vi "monitor registers.vi"(7 "register monitor queue":refnum<queue>, 8 "error in":errorcluster, 9 "Registers":T1[](array[typedef]), 10 "bus instance name":string, 11 "fpga interface in":refnum<k20>) -> (0 "error out":errorcluster, 2 "registers out":string[][](array[string]), 3 "fpga interface out":refnum<k20>, 5 "register monitor queue out":refnum<queue>)   [LabVIEW 2025, in "Automotive Vision.lvclass"]
uses:
  Automotive Vision.lvclass
  Automotive Vision.lvclass/Automotive Vision.ctl
  <instrlib>/FlexRIO/API/Host/v1/NI FlexRIO API v1.lvlib
  regitster_value.ctl
  register.ctl
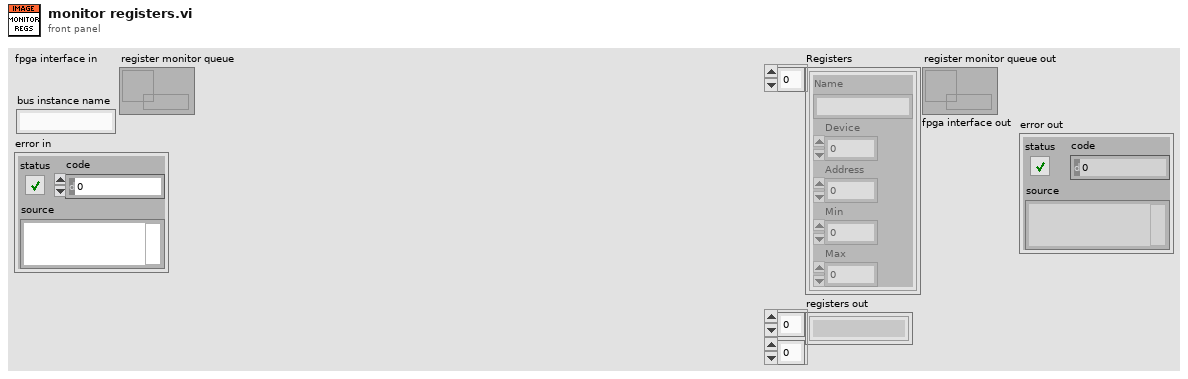
[diagram p1: front panel]
types:
  T1 = typedef "Automotive Vision.lvclass/register.ctl" = cluster{"Name":string, "Device":u8, "Address":u16, "Min":u16, "Max":u16}
  T2 = typedef "Automotive Vision.lvclass/regitster_value.ctl" = cluster{"Source":u8, "Address":u16, "Value":u16}
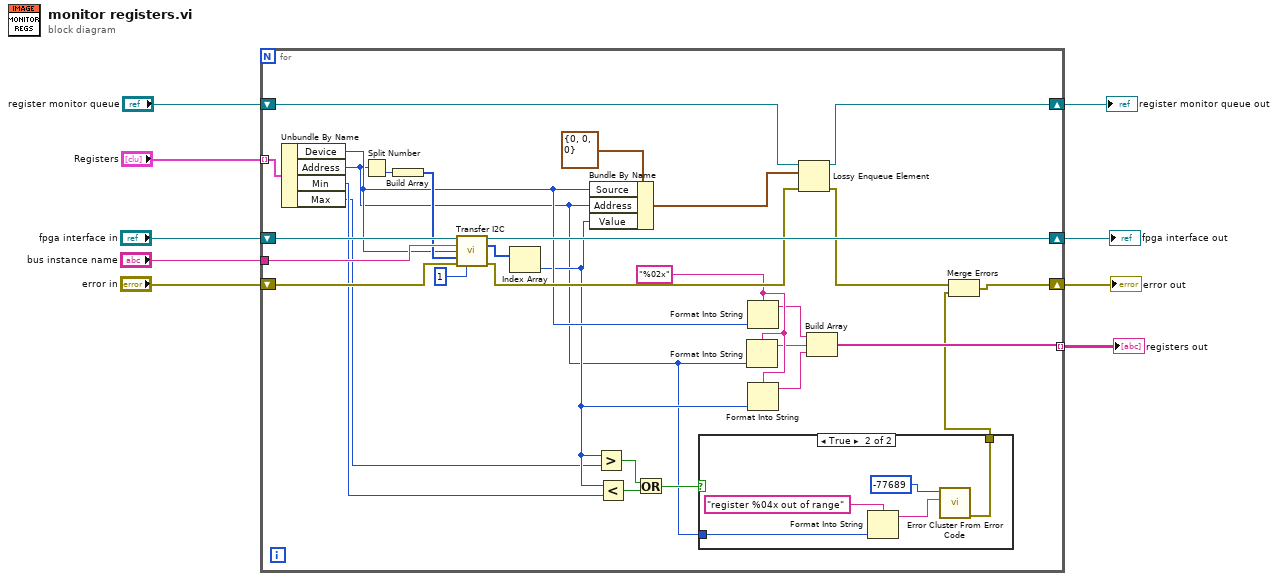
[diagram p0: block diagram]
diagram:
  n1 = for {
    tunnel: "Registers" -> [w39] mode=indexing
    tunnel: "bus instance name" -> [w37]
    shift-right: [w11] -> w2
    shift-left: "error in" -> [w34]
    shift-right: [w32] -> w3
    shift-left: "fpga interface in" -> [w38]
    shift-right: [w27] -> w4
    shift-left: "register monitor queue" -> [w29]
    tunnel: [w20] -> w1 mode=indexing
    w25 = "%02x" ("format string")
    n2 = Unbundle By Name(w39) -> ("Device"=w24:u8, "Address"=w13:u16, "Min"=w19:u16, "Max"=w15:u16)
    n3 = Split Number(x=w13) -> (lo(x)=w36:u8)  [unwired: 1 out]
    n4 = Build Array(w36) -> (w35:u8[])
    n5 = call <instrlib>:"Transfer I2C.vi"("fpga interface in"=w38, "bus instance name"=w37, "slave address"=w24, "write data"=w35, "error in"=w34, "num bytes to read"=u32 1) -> ("fpga interface out"=w32:refnum<k20>, "read data"=w30:u8[], "error out"=w26:errorcluster)  [unwired: 6 in, 1 out]
    n6 = Index Array(array=w30) -> (element=w16:u8)  [unwired: 1 in]
    n7 = Bundle By Name(cluster=T2 {"Source"=0, "Address"=0, "Value"=0} ("Register Value"), "Source"=w24, "Address"=w13, "Value"=w16) -> (w28:T2)
    n8 = Greater?(x=w16, y=w15) -> (0:w17:bool)
    n9 = Less?(x=w16, y=w19) -> (x < y?=w18:bool)
    n10 = Or(x=w17, y=w18) -> (x .or. y?=w14:bool)
    n11 = case shown="True" w14 {
      tunnel: w13 -> [_ w43]
      tunnel: [_ w40] -> w10
      frame False {
      }
      frame True {
        n12 = Format Into String(format string="register %04x out of range" ("error message (\"\")"), w43) -> (resulting string=w42:string)  [unwired: 2 in, 1 out]
        n13 = call <vilib>:"Error Cluster From Error Code.vi"("error message (\"\")"=w42, "error code (0)"=-77689) -> ("error out"=w40:errorcluster)  [unwired: 7 in]
      }
    }
    n14 = Format Into String(format string=w25, w13) -> (resulting string=w23:string)  [unwired: 2 in, 1 out]
    n15 = Format Into String(format string=w25, w24) -> (resulting string=w21:string)  [unwired: 2 in, 1 out]
    n16 = Format Into String(format string=w25, w16) -> (resulting string=w22:string)  [unwired: 2 in, 1 out]
    n17 = Lossy Enqueue Element(queue=w29, element=w28, error in (no error)=w26) -> (queue out=w27:refnum<queue>, error out=w12:errorcluster)  [unwired: 2 out]
    n18 = Build Array(w21, w23, w22) -> (w20:string[])
    n19 = Merge Errors(w12, w10) -> (w11:errorcluster)
  }
  "register monitor queue out" <- w4
  "fpga interface out" <- w3
  "error out" <- w2
  "registers out" <- w1
